vi "Prepare Control.vi"(7 "VolatusAPI":refnum<class "VolatusAPI.lvclass">, 8 "error in (no error)":errorcluster, 11 "ValveControl in":refnum<class "BangBangControl.lvclass">) -> (0 "error out":errorcluster, 3 "ValveControl out":refnum<class "BangBangControl.lvclass">)   [LabVIEW 2020, in "VolatusControl.lvlib" / "BangBangControl.lvclass"]
uses:
  BangBangControl.lvclass
  BangBangControl.lvclass/BangBangControl.ctl
  Volatus/VolatusAPI/VolatusAPI.lvclass
  lv-cdm/CDM-Config/Config Element/Config Element.lvclass
  PV Calc/PV Calc.lvclass
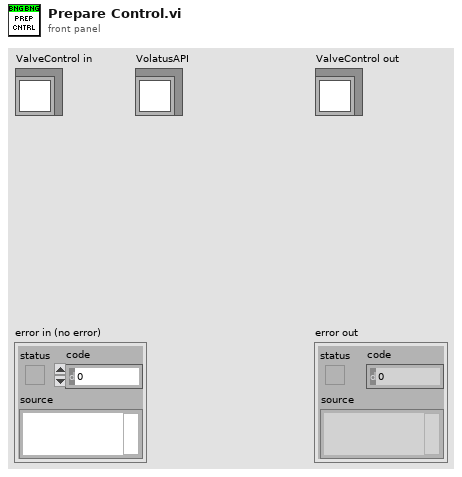
[diagram p1: front panel]
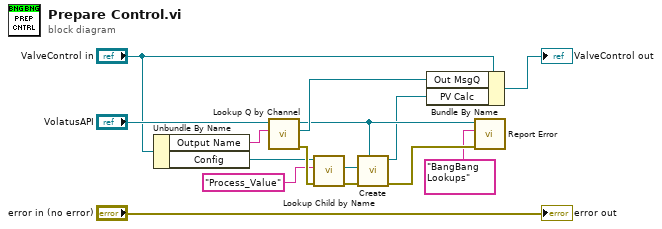
[diagram p0: block diagram]
diagram:
  n1 = Unbundle By Name("ValveControl in") -> ("Output Name"=w12:string, "Config"=w6:refnum<class "Config Element.lvclass">)
  n2 = call "Lookup Q by Channel.vi"("Channel Name"=w12, "VolatusAPI in"="VolatusAPI") -> ("error out"=w14:errorcluster, "MessageQ"=w10:refnum<class "MessageQ.lvclass">, "VolatusAPI out"=w2:refnum<class "VolatusAPI.lvclass">)  [unwired: 7 in]
  n3 = call "Lookup Child by Name.vi"("error in (no error)"=w14, "Name"="Process_Value", "Config Element in"=w6) -> ("error out"=w4:errorcluster, "Child"=w3:refnum<class "Config Element.lvclass">)  [unwired: 5 in, 2 out]
  n4 = call "Create.vi"("VolatusAPI"=w2, "error in (no error)"=w4, "Config Element"=w3) -> ("error out"=w15:errorcluster, "PV Calc out"=w1:refnum<class "PV Calc.lvclass">)  [unwired: 7 in]
  n5 = Bundle By Name(cluster="ValveControl in", "Out MsgQ"=w10, "PV Calc"=w1) -> (→"ValveControl out":refnum<class "BangBangControl.lvclass">)
  n6 = call "Report Error.vi"("error in (no error)"=w15, "Context"="BangBang Lookups", "VolatusAPI in"=w2) -> ()  [unwired: 7 in, 2 out]
  "error out" <- "error in (no error)"
